vi "PicoScope4000aSetRapidSegments.vi"(5 "RapidBlock":bool=TRUE, 7 "nSegments":T1 format="%.4p", 8 "error in (no error)":errorcluster, 11 "handle in":i16) -> (0 "error out":errorcluster, 3 "handle out":i16, 6 "nCaptures":u64)   [LabVIEW 2010]
doc: "Calls ps5000aMemorySegments, and ps5000aSetNoOfCaptures"
uses:
  ps4000a.dll
  shared/nSegments.ctl
panel:
  out "nMaxSamples":u64
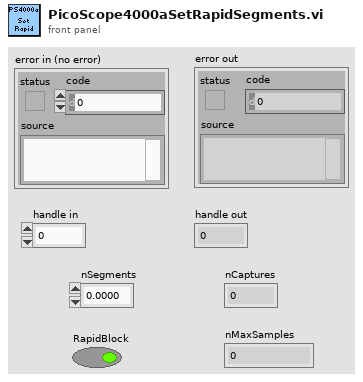
[diagram p1: front panel]
types:
  T1 = typedef "nSegments.ctl" = u64
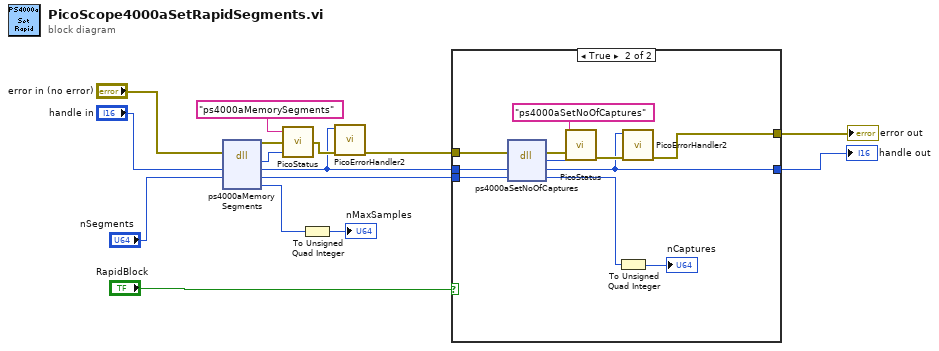
[diagram p0: block diagram]
diagram:
  n1 = dll-call lib="ps4000a.dll" fn="ps4000aMemorySegments" ("ps3000.dll:_ps3000_open_unit@0")(error in="error in (no error)", "handle"="handle in", "nSegments"="nSegments") -> (error out=w14:errorcluster, "PICO_STATUS"=w15:u32, "handle"=w10:i16, "nSegments"=w12:u32, "nMaxSamples"=w1:i32)  [unwired: 3 in, 1 out]
  n2 = call "PicoStatus.vi"("PICO STATUS"=w15, "error in"=w14, "source"="ps4000aMemorySegments") -> ("error out"=w11:errorcluster)
  n3 = To Unsigned Quad Integer(1:w1) -> (0:→"nMaxSamples":u64)
  n4 = call "PicoErrorHandler2.vi"("error in (no error)"=w11, "handle In"=w10) -> ("error out"=w9:errorcluster)  [unwired: 9 in]
  n5 = case shown="True" "RapidBlock" {
    tunnel: w12 -> [_ w28]
    tunnel: w10 -> [w16 w25]
    tunnel: w9 -> [w17 w22]
    tunnel: [w17 w21] -> w6
    tunnel: [w16 w20] -> w5
    frame False {
    }
    frame True {
      n6 = dll-call lib="ps4000a.dll" fn="ps4000aSetNoOfCaptures" ("ps3000.dll:_ps3000_open_unit@0")(error in=w22, "handle"=w25, "nCaptures"=w28) -> (error out=w27:errorcluster, "PICO_STATUS"=w23:u32, "handle"=w20:i16, "nCaptures"=w18:u32)  [unwired: 2 in, 1 out]
      n7 = call "PicoStatus.vi"("PICO STATUS"=w23, "error in"=w27, "source"="ps4000aSetNoOfCaptures") -> ("error out"=w24:errorcluster)
      n8 = To Unsigned Quad Integer(1:w18) -> (0:→"nCaptures":u64)
      n9 = call "PicoErrorHandler2.vi"("error in (no error)"=w24, "handle In"=w20) -> ("error out"=w21:errorcluster)  [unwired: 9 in]
    }
  }
  "error out" <- w6
  "handle out" <- w5
